vi "Collect.vi"(8 "error in (no error)":errorcluster, 11 "Session Handle in":T1) -> (0 "error out":errorcluster, 2 "Metrics":refnum<data-value>[](array[refnum]), 3 "Session Handle out":T1)   [LabVIEW 2020, in "Registry.lvlib" / "Registry Session.lvclass"]
uses:
  Registry Session.lvclass
  Typedefs/Session Handle.ctl
  metrics/metric/Metric.lvclass
  Registry Session.lvclass/Registry Session.ctl
  collector/collectable/Collectable.lvclass
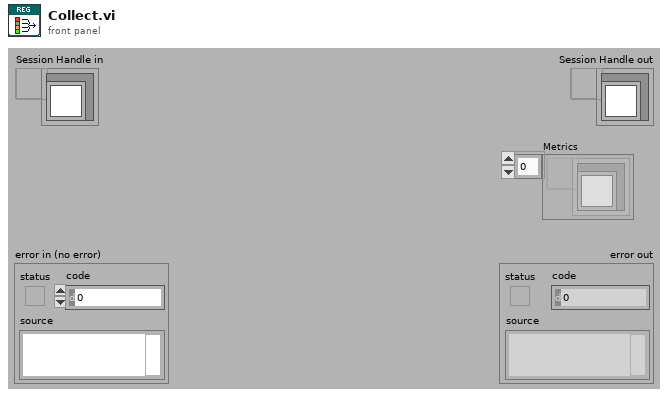
[diagram p1: front panel]
types:
  T1 = typedef "Registry.lvlib/Registry Session.lvclass/Session Handle.ctl" = refnum<data-value>
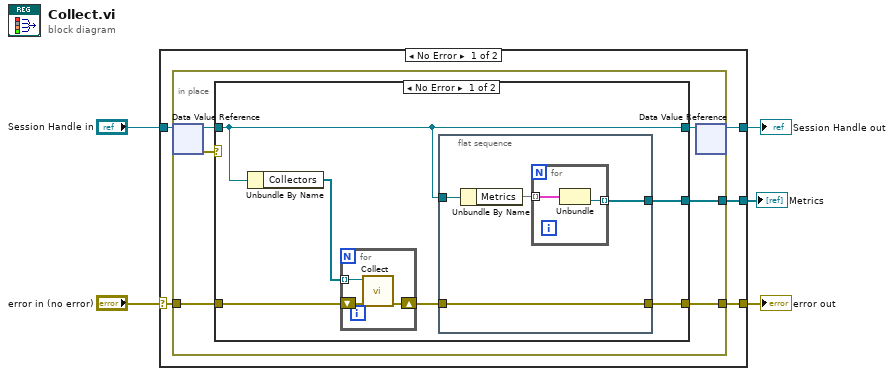
[diagram p0: block diagram]
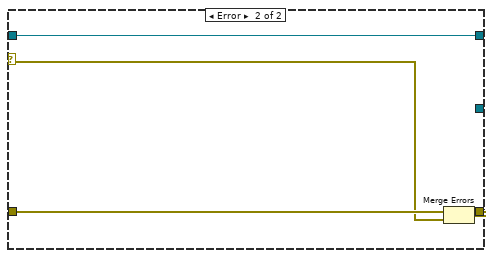
[diagram p2: hidden frame]
diagram:
  n1 = case shown="No Error" "error in (no error)" {
    selector: "error in (no error)" -> [w8 w36]
    tunnel: "Session Handle in" -> [w10 w37]
    tunnel: [w9 w37] -> w4
    tunnel: [w7 w36] -> w3
    tunnel: [w6 _] -> w1
    frame No Error {
      n2 = in-place {
        in-place-border: w8 -> [w12]
        in-place-border: [w15] -> w7
        in-place-border: [w11] -> w6
        n3 = in-place-dvr #1(w10) -> (w16:refnum<class "Registry Session.lvclass">, w13:errorcluster)
        n4 = case shown="No Error" w13 {
          selector: w13 -> [_ w34]
          tunnel: w16 -> [w19 w32]
          tunnel: [w17 w33] -> w15
          tunnel: [w19 w32] -> w14
          tunnel: w12 -> [w20 w35]
          tunnel: [w22 _] -> w11
          frame No Error {
            n5 = Unbundle By Name(w19) -> ("Collectors"=w21:refnum<class "Collectable.lvclass">[])
            n6 = for {
              tunnel: w21 -> [w31] mode=indexing
              shift-right: [w29] -> w18
              shift-left: w20 -> [w30]
              n7 = call-dynamic "Collect.vi"("error in (no error)"=w30, "Collectable in"=w31) -> ("error out"=w29:errorcluster)  [unwired: 7 in, 2 out]
            }
            n8 = flat-sequence {
              tunnel: [w26] -> w22
              tunnel: w19 -> [w25]
              tunnel: w18 -> [w23]
              tunnel: [w23] -> w17
              frame #0 {
                n9 = Unbundle By Name(w25) -> ("Metrics"=w24:map{string, refnum<data-value>})
                n10 = for {
                  tunnel: [w28] -> w26 mode=indexing
                  tunnel: w24 -> [w27] mode=indexing
                  n11 = Unbundle(w27) -> ("Metric"=w28:refnum<data-value>)  [unwired: 1 out]
                }
              }
            }
          }
          frame Error {
            n12 = Merge Errors(w35, w34) -> (w33:errorcluster)
          }
        }
        n13 = in-place-dvr #1(w14) -> (w9:T1)  [unwired: 1 out]
      }
    }
    frame Error {
    }
  }
  "Session Handle out" <- w4
  "error out" <- w3
  "Metrics" <- w1
